vi "NUEVA PRUEBA SUPER OFICIAL NO FAKE.vi"() -> ()   [LabVIEW 2019]
uses:
  <vilib>/myRIO/Common/Instrument Driver Framework/myRIO v1.0/Encoder/typedefs/Encoder Signal Mode.ctl
  <vilib>/myRIO/Common/Instrument Driver Framework/myRIO v1.0/Encoder/typedefs/Encoder Configuration v1.0.ctl
  <vilib>/myRIO/Instrument Drivers/Onboard IO/Encoder/typedefs/Encoder Reference.ctl
  <vilib>/myRIO/Common/Instrument Driver Framework/Utilities/typedefs/myRIO Generic Hardware Reference.ctl
  <vilib>/myRIO/Common/Instrument Driver Framework/Utilities/typedefs/Hardware Version Enum.ctl
  <vilib>/myRIO/Common/Instrument Driver Framework/Utilities/typedefs/myRIO v1.0 Reference.ctl
  <vilib>/myRIO/Common/Instrument Driver Framework/Utilities/typedefs/Generic FPGA Reference.ctl
  <vilib>/myRIO/Common/Instrument Driver Framework/myRIO v1.0/Encoder/typedefs/Encoder Channels Enum.ctl
  <vilib>/userDefined/High Color/nirio_resource_hc.ctl
  <vilib>/myRIO/Instrument Drivers/Onboard IO/DIO/typedefs/DIO Reference.ctl
  <vilib>/myRIO/Common/Instrument Driver Framework/myRIO v1.0/DIO/typedefs/DIO Channels List.ctl
  <vilib>/myRIO/Common/Instrument Driver Framework/myRIO v1.0/DIO/typedefs/DIO Channels Enum.ctl
  <vilib>/myRIO/Instrument Drivers/Onboard IO/PWM/typedefs/PWM Reference.ctl
  <vilib>/myRIO/Common/Instrument Driver Framework/myRIO v1.0/PWM/typedefs/PWM Channels Enum.ctl
  <vilib>/myRIO/Instrument Drivers/Onboard IO/PWM/typedefs/PWM Configuration.ctl
  <vilib>/myRIO/Common/Instrument Driver Framework/myRIO v1.0/Encoder/vis/myRIO v1.1 Open Encoder.vi
  <vilib>/myRIO/Common/Instrument Driver Framework/Utilities/vis/Is FPGA Ref Available.vi
  <vilib>/myRIO/Common/Instrument Driver Framework/myRIO v1.0/DIO/vis/myRIO v1.1 Open DIO.vi
  <vilib>/myRIO/Instrument Drivers/Onboard IO/DIO/vis/Write.vi
  <vilib>/myRIO/Common/Instrument Driver Framework/myRIO v1.0/PWM/vis/myRIO v1.1 Open PWM.vi
  <vilib>/myRIO/Instrument Drivers/Onboard IO/PWM/vis/Set Duty Cycle and Frequency.vi
  <vilib>/myRIO/Common/Instrument Driver Framework/Utilities/vis/Validate Channels.vi
  <vilib>/myRIO/Common/Instrument Driver Framework/myRIO v1.0/Encoder/vis/myRIO v1.0 Reserve Encoder.vi
  <vilib>/myRIO/Common/Instrument Driver Framework/myRIO v1.0/DIO/vis/myRIO v1.0 Reserve DIO.vi
  <vilib>/myRIO/Common/Instrument Driver Framework/myRIO v1.0/PWM/vis/myRIO v1.0 Reserve PWM.vi
  <vilib>/myRIO/Common/Instrument Driver Framework/myRIO v1.0/Encoder/vis/myRIO v1.0 Close Encoder.vi
  <vilib>/myRIO/Common/Instrument Driver Framework/myRIO v1.0/Encoder/vis/myRIO v1.0 Build MUX Configuration Encoder.vi
  <vilib>/myRIO/Common/Instrument Driver Framework/myRIO v1.0/Resource Manager/vis/myRIO v1.0 Reserve Channel List.vi
  <vilib>/myRIO/Common/Instrument Driver Framework/myRIO v1.0/DIO/vis/myRIO v1.0 Build MUX Configuration DIO.vi
  <vilib>/myRIO/Common/Instrument Driver Framework/myRIO v1.0/PWM/vis/myRIO v1.0 Build MUX Configuration PWM.vi
  <vilib>/myRIO/Common/Instrument Driver Framework/myRIO v1.0/Encoder/vis/myRIO v1.0 Unreserve Encoder.vi
  <vilib>/myRIO/Common/Instrument Driver Framework/myRIO v1.0/Resource Manager/vis/myRIO v1.0 Create Configuration List.vi
  <vilib>/myRIO/Common/Instrument Driver Framework/myRIO v1.0/Resource Manager/vis/myRIO v1.0 Reserve Channel.vi
  <vilib>/myRIO/Common/Instrument Driver Framework/myRIO v1.0/Resource Manager/vis/myRIO v1.0 Unreserve Channel.vi
  <vilib>/myRIO/Common/Instrument Driver Framework/myRIO v1.0/Resource Manager/vis/myRIO v1.0 Unreserve Channel List.vi
  <vilib>/myRIO/Common/Instrument Driver Framework/myRIO v1.0/Resource Manager/vis/myRIO v1.0 Build Mutex Name.vi
  <vilib>/Utility/VariantDataType/GetNumericInfo.vi
  <vilib>/Utility/error.llb/Error Cluster From Error Code.vi
  <vilib>/myRIO/Common/Instrument Driver Framework/myRIO v1.0/myRIO v1.1 Open.vi
  <vilib>/myRIO/Common/Instrument Driver Framework/Utilities/vis/IO Manager.vi
  <vilib>/myRIO/Common/Instrument Driver Framework/Utilities/vis/Configuration Manager.vi
  <vilib>/myRIO/Common/Instrument Driver Framework/myRIO v1.0/Resource Manager/vis/myRIO v1.0 Configure IO.vi
  <vilib>/myRIO/Common/Instrument Driver Framework/myRIO v1.0/myRIO v1.0 Close.vi
  <vilib>/myRIO/Common/Instrument Driver Framework/myRIO v1.0/Encoder/vis/myRIO v1.0 Configure Encoder.vi
  <vilib>/myRIO/Common/Instrument Driver Framework/myRIO v1.0/Encoder/vis/myRIO v1.0 Enable Encoder.vi
  <vilib>/myRIO/Common/Instrument Driver Framework/myRIO v1.0/Encoder/vis/myRIO v1.0 Read Encoder.vi
  <vilib>/myRIO/Common/Instrument Driver Framework/myRIO v1.0/DIO/vis/myRIO v1.0 Write DIO.vi
  <vilib>/myRIO/Common/Instrument Driver Framework/myRIO v1.0/PWM/vis/myRIO v1.0 Write PWM.vi
  <vilib>/myRIO/Common/Instrument Driver Framework/myRIO v1.0/Encoder/vis/myRIO v1.0 Shutdown Encoder.vi
  <vilib>/myRIO/Instrument Drivers/Onboard IO/Encoder/vis/myRIO Encoder Open.xnode
  <vilib>/myRIO/Express VI/Onboard IO/DO/DO Express VI.xnode
  <vilib>/myRIO/Instrument Drivers/Onboard IO/DIO/vis/myRIO DIO Open.xnode
  <vilib>/myRIO/Express VI/Onboard IO/PWM/PWM Express VI.xnode
  <vilib>/myRIO/Instrument Drivers/Onboard IO/PWM/vis/myRIO PWM Open.xnode
  <vilib>/myRIO/Instrument Drivers/Onboard IO/PWM/PWM.lvlib
  <vilib>/myRIO/Instrument Drivers/Onboard IO/DIO/DIO.lvlib
  <vilib>/myRIO/Instrument Drivers/Onboard IO/Encoder/Encoder.lvlib
panel:
  in  "RESET_GENERAL":bool
  out "Grafico_Trayectoria_XY":cluster{"X":dbl, "Y":dbl}[](graph)
  out "Grafico_Orientacion_rad":dbl(graph)
  out "Grafico_Posicion_X":dbl(graph)
  out "Auto_Stop_Giro_360":bool
  out "Objetivo_360_Alcanzado":bool
  in  "Modo_Auto_Giro_360":bool
  out "Auto_Stop_General":bool
  out "Auto_Stop_50cm":bool
  out "Objetivo_50cm_Alcanzado":bool
  in  "Modo_Auto_50cm":bool
  in  "Distancia_Objetivo_m":dbl=0.25 format="%#_13g"
  out "Stop_25cm_Memorizado":bool
  out "Auto_Stop_25cm":bool
  in  "Modo_Auto_25cm":bool
  out "Objetivo_25cm_Alcanzado":bool
  out "Y_Actual_m":dbl
  out "X_Actual_m":dbl
  out "Delta_Y_m":dbl
  out "Delta_X_m":dbl
  out "Theta_Medio_rad":dbl
  out "Theta_Acumulado_rad":dbl
  out "Delta_theta_rad":dbl
  out "Delta_s_Centro_m":dbl
  out "Delta_s_Der_m":dbl
  out "Delta_s_Izq_m":dbl
  out "Tiempo_Valido":bool
  out "Delta_t_validado":dbl
  out "Delta_t_ms":u32
  out "Delta_N_Der":dbl
  out "Delta_N_Izq":dbl
  out "Encoder_Der_Count":i32=-24622
  out "Encoder_Izq_Count":i32=30472
  in  "Duty Cycle (%)":dbl
  in  "Enum":T1(ring)
  in  "stop":bool
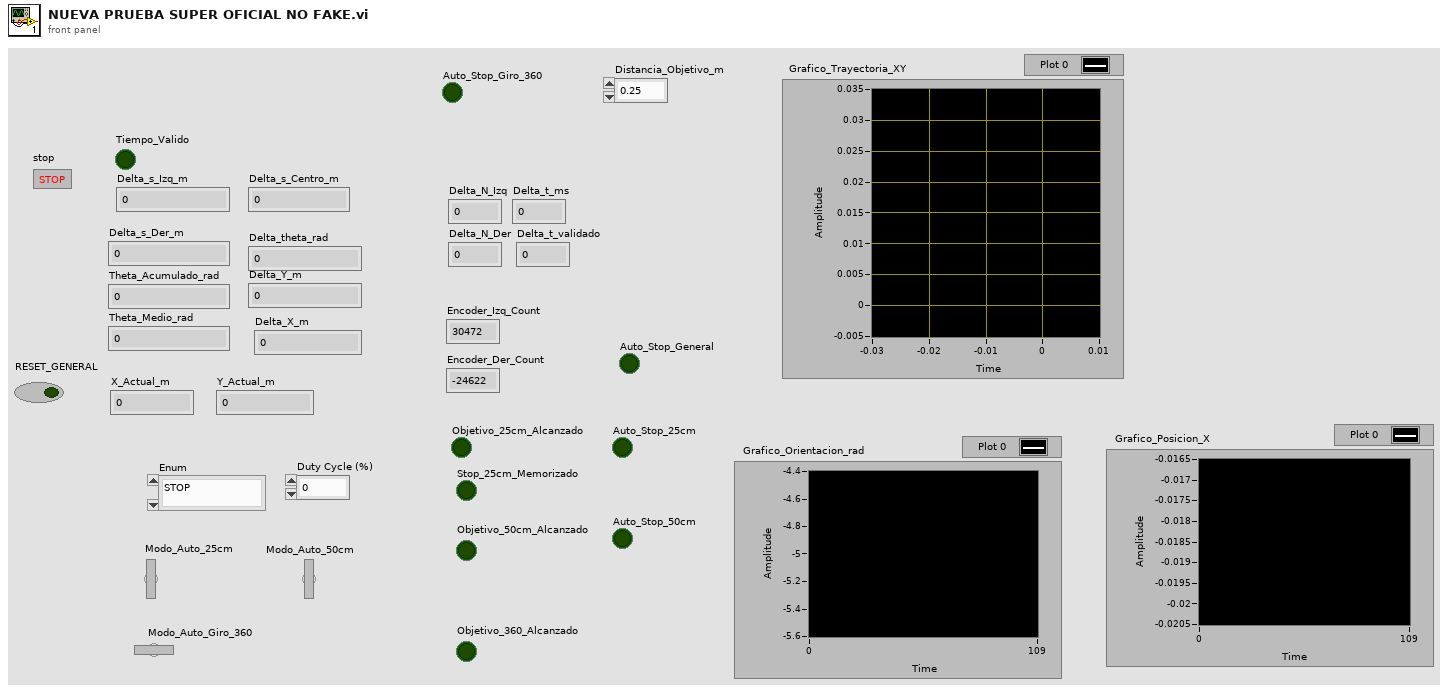
[diagram p1: front panel]
types:
  T1 = enum16{"STOP", "ADELANTE", "ATRÁS", "GIRO_IZQ", "GIRO_DER"}
  T2 = typedef "Encoder Signal Mode.ctl" = enum16{"Quadrature phase signal", "Step and direction signal"}
  T3 = typedef "Encoder.lvlib/Encoder Reference.ctl" = cluster{"myRIO Reference":T4, "Encoder Channels Enum":T8}
  T4 = typedef "myRIO Generic Hardware Reference.ctl" = cluster{"myRIO Model":T5, "myRIO Hardware Reference":T6}
  T5 = typedef "Hardware Version Enum.ctl" = enum16{"Unknown", "myRIO-1900", "myRIO-1950", "roboRIO", "NI ELVIS RIO CM", "ELVIS III"}
  T6 = typedef "myRIO v1.0 Reference.ctl" = cluster{"Generic FPGA Reference":T7, "Allow multiple opens":bool}
  T7 = typedef "Generic FPGA Reference.ctl" = refnum<k20>
  T8 = typedef "Encoder Channels Enum.ctl" = enum16{"Not Connected", "C/ENC0", "C/ENC1", "A/ENC", "A/ENC0", "A/ENC1", "A/ENC2", "A/ENC3", "A/ENC4", "A/ENC5", "A/ENC6", "A/ENC7", "A/ENC8", "A/ENC9", "B/ENC", "B/ENC0", "B/ENC1", "B/ENC2", "B/ENC3", "B/ENC4", "B/ENC5", "B/ENC6", "B/ENC7", "B/ENC8", "B/ENC9", "DIO/ENC0", "DIO/ENC1", "DIO/ENC2", "DIO/ENC3", "DIO/ENC4"}
  T9 = typedef "DIO.lvlib/DIO Reference.ctl" = cluster{"myRIO Reference":T4, "DIO Channels List":T10}
  T10 = typedef "DIO Channels List.ctl" = T11[]
  T11 = typedef "DIO Channels Enum.ctl" = enum16{"Not Connected", "C/DIO0", "C/DIO1", "C/DIO2", "C/DIO3", "C/DIO4", "C/DIO5", "C/DIO6", "C/DIO7", "A/DIO0", "A/DIO1", "A/DIO2", "A/DIO3", "A/DIO4", "A/DIO5", "A/DIO6", "A/DIO7", "A/DIO8", "A/DIO9", "A/DIO10", "A/DIO11", "A/DIO12", "A/DIO13", "A/DIO14", "A/DIO15", "A/DIO16", "A/DIO17", "A/DIO18", "A/DIO19", "B/DIO0", "B/DIO1", "B/DIO2", "B/DIO3", "B/DIO4", "B/DIO5", "B/DIO6", "B/DIO7", "B/DIO8", "B/DIO9", "B/DIO10", "B/DIO11", "B/DIO12", "B/DIO13", "B/DIO14", "B/DIO15", "B/DIO16", "B/DIO17", "B/DIO18", "B/DIO19", "LED0", "LED1", "LED2", "LED3", "Button0", "DIO/DIO0", "DIO/DIO1", "DIO/DIO2", "DIO/DIO3", "DIO/DIO4", "DIO/DIO5", "DIO/DIO6", "DIO/DIO7", "DIO/DIO8", "DIO/DIO9", "SPI/CS0", "SPI/CS1", "SPI/CS2", "SPI/CS3", "LED RADIO (Green)", "LED RADIO (Red)", "LED COMM (Green)", "LED COMM (Red)", "LED MODE (Green)", "LED MODE (Red)"}
  T12 = typedef "nirio_resource_hc.ctl" = tag
  T13 = typedef "PWM.lvlib/PWM Reference.ctl" = cluster{"myRIO Reference":T4, "PWM Channels Enum":T14, "PWM Configuration":T15}
  T14 = typedef "PWM Channels Enum.ctl" = enum16{"Not Connected", "C/PWM0", "C/PWM1", "A/PWM0", "A/PWM1", "A/PWM2", "A/PWM3", "A/PWM4", "A/PWM5", "A/PWM6", "A/PWM7", "A/PWM8", "A/PWM9", "A/PWM10", "A/PWM11", "A/PWM12", "A/PWM13", "A/PWM14", "A/PWM15", "A/PWM16", "A/PWM17", "A/PWM18", "A/PWM19", "B/PWM0", "B/PWM1", "B/PWM2", "B/PWM3", "B/PWM4", "B/PWM5", "B/PWM6", "B/PWM7", "B/PWM8", "B/PWM9", "B/PWM10", "B/PWM11", "B/PWM12", "B/PWM13", "B/PWM14", "B/PWM15", "B/PWM16", "B/PWM17", "B/PWM18", "B/PWM19", "PWM/PWM0", "PWM/PWM1", "PWM/PWM2", "PWM/PWM3", "PWM/PWM4", "PWM/PWM5", "PWM/PWM6", "PWM/PWM7", "PWM/PWM8", "PWM/PWM9"}
  T15 = typedef "PWM.lvlib/PWM Configuration.ctl" = cluster{"Frequency":dbl, "Duty Cycle":dbl}
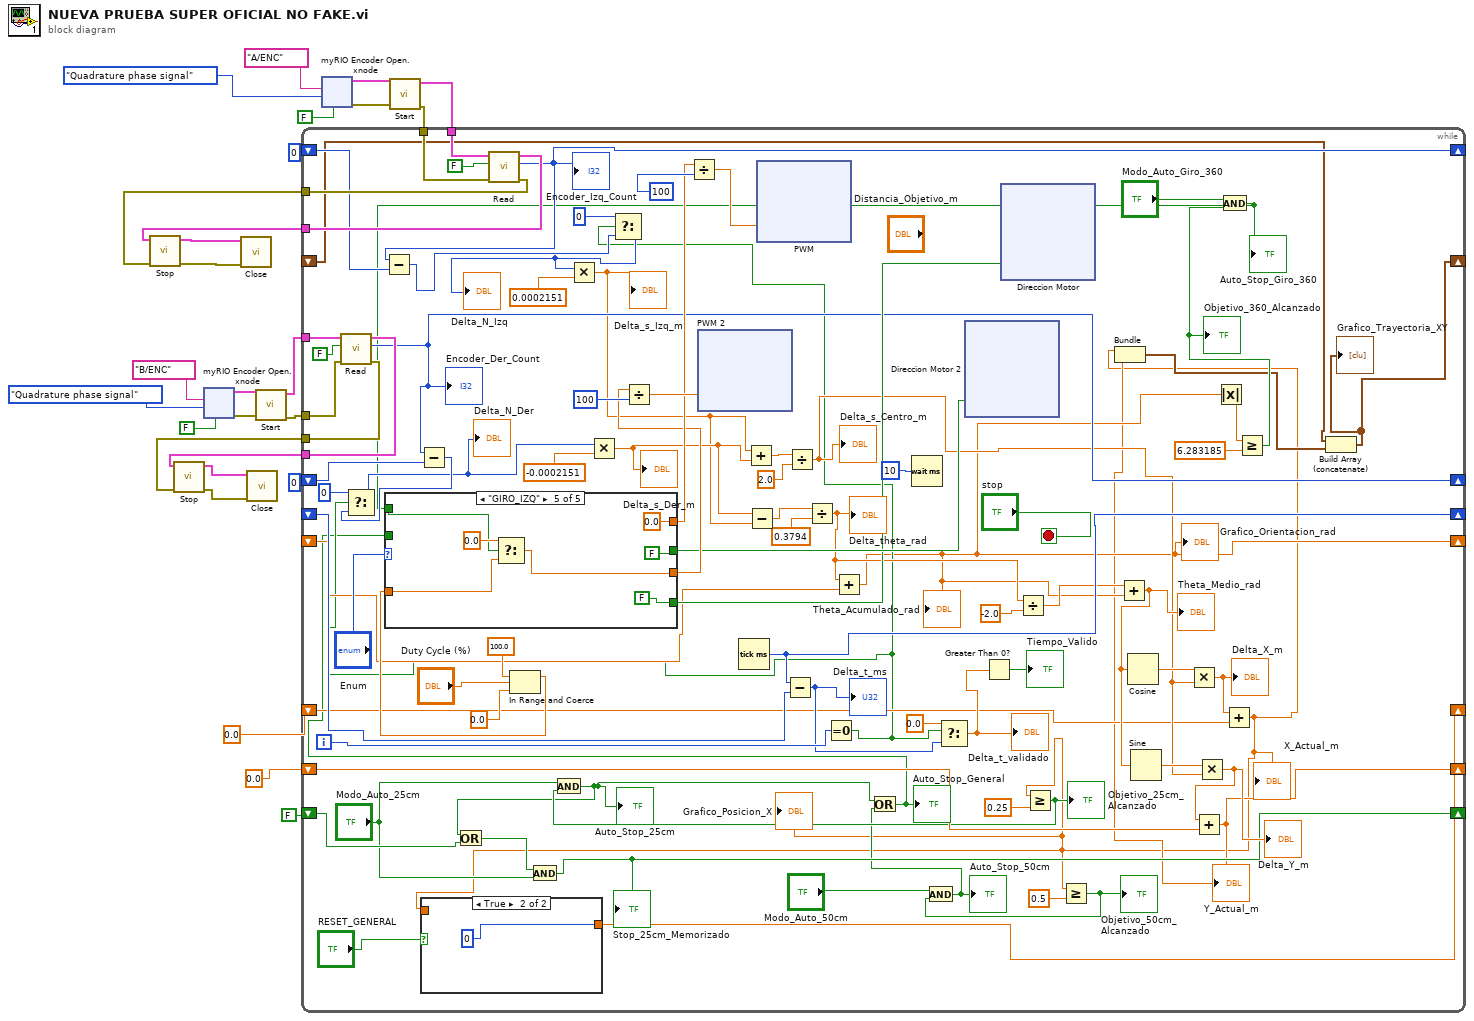
[diagram p0: block diagram]
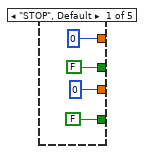
[diagram p3: hidden frame]
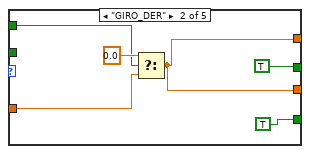
[diagram p4: hidden frame]
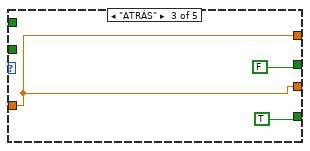
[diagram p5: hidden frame]
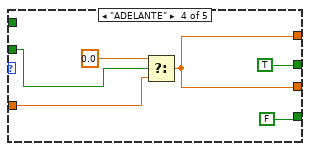
[diagram p6: hidden frame]
diagram:
  n1 = xnode "myRIO Encoder Open.xnode"("Channel Name"=tag "B/ENC", "Start Counter"=FALSE, "Encoder Signal Mode"=Encoder_Signal_Mode."Quadrature phase signal") -> ("error out"=w12:errorcluster, "Encoder Ref Out"=w13:T3)  [unwired: 2 in]
  n2 = call <vilib>:"Start.vi"("error in (no error)"=w12, "Encoder Ref In"=w13) -> ("error out"=w10:errorcluster, "Encoder Ref Out"=w11:T3)  [unwired: 8 in]
  n3 = xnode "myRIO Encoder Open.xnode"("Channel Name"=tag "A/ENC", "Start Counter"=FALSE, "Encoder Signal Mode"=Encoder_Signal_Mode."Quadrature phase signal") -> ("error out"=w23:errorcluster, "Encoder Ref Out"=w24:T3)  [unwired: 2 in]
  n4 = call <vilib>:"Start.vi"("error in (no error)"=w23, "Encoder Ref In"=w24) -> ("error out"=w21:errorcluster, "Encoder Ref Out"=w22:T3)  [unwired: 8 in]
  n5 = while {
    tunnel: w22 -> [w100]
    tunnel: w21 -> [w99]
    tunnel: [w97] -> w20
    tunnel: [w96] -> w19
    tunnel: w11 -> [w95]
    tunnel: w10 -> [w93]
    tunnel: [w92] -> w9
    tunnel: [w91] -> w8
    shift-right: [w90] -> _
    shift-left: 0 ("Counter Value") -> [w89]
    shift-right: [w87] -> _
    shift-left: 0 ("Counter Value") -> [w88]
    shift-right: [w86] -> _
    shift-left: _ -> [w85]
    shift-right: [w35] -> _
    shift-left: _ -> [w71]
    shift-right: [w29] -> _
    shift-left: 0.0 -> [w62]
    shift-right: [w34] -> _
    shift-left: 0.0 -> [w60]
    shift-right: [w48] -> _
    shift-left: FALSE -> [w51]
    shift-right: [w31] -> _
    shift-left: _ -> [w32]
    i -> [w83]
    stop <- "stop" stop-if-true
    n6 = call <vilib>:"Read.vi"("error in (no error)"=w93, "Reset Counter"=FALSE, "Encoder Ref In"=w95) -> ("error out"=w91:errorcluster, "Counter Value"=w87:i32, "Encoder Ref Out"=w92:T3)  [unwired: 4 in, 2 out]
    "Encoder_Der_Count" <- w87
    n7 = Subtract(x=w87, y=w88) -> (x-y=w54:i32)
    n8 = call <vilib>:"Read.vi"("error in (no error)"=w99, "Reset Counter"=FALSE, "Encoder Ref In"=w100) -> ("error out"=w96:errorcluster, "Counter Value"=w90:i32, "Encoder Ref Out"=w97:T3)  [unwired: 4 in, 2 out]
    "Encoder_Izq_Count" <- w90
    n9 = Subtract(x=w90, y=w89) -> (x-y=w58:i32)
    n10 = In Range and Coerce(upper limit=100.0, x="Duty Cycle (%)", lower limit=0.0) -> (coerced(x)=w101:dbl)  [unwired: 1 out]
    n11 = Tick Count (ms)() -> (millisecond timer value=w86:u32)
    n12 = Subtract(x=w86, y=w85) -> (x-y=w82:u32)
    "Delta_t_ms" <- w82
    n13 = Equal To 0?(x=w83) -> (x = 0?=w55:bool)
    n14 = Select(t=0, s=w55, f=w54) -> (s? t:f=w53:i32)
    "Delta_N_Der" <- w53
    n15 = Multiply(x=w53, y=-0.0002151) -> (x*y=w75:dbl)
    "Delta_s_Der_m" <- w75
    n16 = Select(t=0, s=w55, f=w58) -> (s? t:f=w57:i32)
    "Delta_N_Izq" <- w57
    n17 = Multiply(x=w57, y=0.0002151) -> (x*y=w74:dbl)
    "Delta_s_Izq_m" <- w74
    n18 = Add(x=w74, y=w75) -> (x+y=w77:dbl)
    n19 = Subtract(x=w75, y=w74) -> (x-y=w73:dbl)
    n20 = Divide(x=w77, y=2.0) -> (x/y=w64:dbl)
    "Delta_s_Centro_m" <- w64
    n21 = Divide(x=w73, y=0.3794) -> (x/y=w70:dbl)
    "Delta_theta_rad" <- w70
    n22 = Add(x=w70, y=w71) -> (x+y=w35:dbl)
    "Theta_Acumulado_rad" <- w35
    "Grafico_Orientacion_rad" <- w35
    n23 = Wait (ms)(milliseconds to wait=10) -> ()  [unwired: 1 out]
    n24 = Select(t=0.0, s=w55, f=w82) -> (s? t:f=w81:dbl)
    "Delta_t_validado" <- w81
    n25 = Greater Than 0?(x=w81) -> (x > 0?=→"Tiempo_Valido":bool)
    n26 = Divide(x=w70, y=-2.0) -> (x/y=w68:dbl)
    n27 = Add(x=w68, y=w35) -> (x+y=w65:dbl)
    "Theta_Medio_rad" <- w65
    n28 = Cosine(x=w65) -> (cos(x)=w67:dbl)
    n29 = Sine(x=w65) -> (sin(x)=w66:dbl)
    n30 = Multiply(x=w67, y=w64) -> (x*y=w63:dbl)
    "Delta_X_m" <- w63
    n31 = Multiply(x=w66, y=w64) -> (x*y=w61:dbl)
    "Delta_Y_m" <- w61
    n32 = Add(x=w61, y=w60) -> (x+y=w34:dbl)
    "Y_Actual_m" <- w34
    n33 = Absolute Value(x=w35) -> (abs(x)=w40:dbl)
    n34 = Add(x=w63, y=w62) -> (x+y=w28:dbl)
    "X_Actual_m" <- w28
    "Grafico_Posicion_X" <- w28
    n35 = case shown="True" "RESET_GENERAL" {
      tunnel: w28 -> [w116 _]
      tunnel: [w116 0] -> w29
      frame False {
      }
      frame True {
      }
    }
    n36 = Greater Or Equal?(x=w28, y=0.25) -> (x >= y?=w52:bool)
    "Objetivo_25cm_Alcanzado" <- w52
    n37 = And(x="Modo_Auto_25cm", y=w52) -> (x .and. y?=w42:bool)
    "Auto_Stop_25cm" <- w42
    n38 = Or(x=w42, y=w51) -> (x .or. y?=w49:bool)
    n39 = And(x=w49, y="Modo_Auto_25cm") -> (x .and. y?=w48:bool)
    "Stop_25cm_Memorizado" <- w48
    n40 = Greater Or Equal?(x=w28, y=0.5) -> (x >= y?=w45:bool)
    "Objetivo_50cm_Alcanzado" <- w45
    n41 = And(x="Modo_Auto_50cm", y=w45) -> (x .and. y?=w44:bool)
    "Auto_Stop_50cm" <- w44
    n42 = Or(x=w42, y=w44) -> (x .or. y?=w41:bool)
    "Auto_Stop_General" <- w41
    n43 = Bundle(w28, w34) -> (w33:cluster{dbl, dbl})  [unwired: 1 in]
    n44 = Greater Or Equal?(x=w40, y=6.283185) -> (x >= y?=w37:bool)
    "Objetivo_360_Alcanzado" <- w37
    n45 = And(x="Modo_Auto_Giro_360", y=w37) -> (x .and. y?=w36:bool)
    "Auto_Stop_Giro_360" <- w36
    n46 = case shown="\"GIRO_IZQ\"" "Enum" {
      tunnel: [FALSE TRUE FALSE TRUE FALSE] -> w106
      tunnel: [0 w122 w128 w131 0.0 ("upper limit")] -> w108
      tunnel: [0 w122 w128 w131 w138] -> w107
      tunnel: [FALSE TRUE TRUE FALSE FALSE] -> w105
      tunnel: w101 -> [_ w123 w128 w132 w139]
      tunnel: w41 -> [_ _ _ w133 _]
      tunnel: w36 -> [_ w124 _ _ w140]
      frame "STOP", Default {
      }
      frame "GIRO_DER" {
        n47 = Select(t=0.0, s=w124, f=w123) -> (s? t:f=w122:dbl)
      }
      frame "ATRÁS" {
      }
      frame "ADELANTE" {
        n48 = Select(t=0.0, s=w133, f=w132) -> (s? t:f=w131:dbl)
      }
      frame "GIRO_IZQ" {
        n49 = Select(t=0.0, s=w140, f=w139) -> (s? t:f=w138:dbl)
      }
    }
    n50 = Divide(x=w107, y=100) -> (x/y=w112:dbl)
    n51 = Divide(x=w108, y=100) -> (x/y=w114:dbl)
    n52 = xnode "PWM 2"("Duty Cycle"=w112) -> ()  [unwired: 1 in, 1 out]
    n53 = xnode "PWM"("Duty Cycle"=w114) -> ()  [unwired: 1 in, 1 out]
    n54 = xnode "Direccion Motor 2"("A/DIO0 (Pin 11)"=w106) -> ()  [unwired: 1 in, 1 out]
    n55 = xnode "Direccion Motor"("B/DIO0 (Pin 11)"=w105) -> ()  [unwired: 1 in, 1 out]
    n56 = Build Array (concatenate)(w32, w33) -> (w31:cluster{dbl, dbl}[])
    "Grafico_Trayectoria_XY" <- w31
  }
  n57 = call <vilib>:"Stop.vi"("error in (no error)"=w19, "Encoder Ref In"=w20) -> ("error out"=w17:errorcluster, "Encoder Ref Out"=w18:T3)  [unwired: 8 in]
  n58 = call <vilib>:"Stop.vi"("error in (no error)"=w8, "Encoder Ref In"=w9) -> ("error out"=w6:errorcluster, "Encoder Ref Out"=w7:T3)  [unwired: 8 in]
  n59 = call <vilib>:"Close.vi"("error in (no error)"=w17, "Encoder Ref In"=w18) -> ()  [unwired: 9 in, 1 out]
  n60 = call <vilib>:"Close.vi"("error in (no error)"=w6, "Encoder Ref In"=w7) -> ()  [unwired: 9 in, 1 out]
